vi "Demo_PlotMusic.vi"() -> ()   [LabVIEW 2021, in "RocketPlotDemo.lvlib"]
uses:
  Demo/RocketPlotDemo.lvlib
  TypeDefs/plot load data V2.ctl
  TypeDefs/plot properties V2.ctl
  TypeDefs/plot attributes V2.ctl
  TypeDefs/Plot scale axis properties.ctl
  TypeDefs/Plot general properties.ctl
  Classes/RocketPlotHandle/SubVIs/Init Options.ctl
  TypeDefs/TimeZone.ctl
  <vilib>/sound2/lvsound2.llb/Sampling Mode.ctl
  Classes/RocketPlotPanel/RocketPlotPanel.lvclass/RocketPlotPanel.ctl
  Classes/BjusticePlotHandle/BjusticePlotHandle.lvclass/BjusticePlotHandle.ctl
  4dfea61d-788a-4186-b191-4cde70d6fed2.vi
  966c8643-725a-46bd-9dd0-b91467cf4ddd.vi
  eb0507fd-03f2-4275-8513-22fa9a77d05c.vi
  2cc444ce-eb93-4e53-95b9-bbf802b1ec09.vi
  0323ff41-b8ad-4ed8-8c31-07cadd3001fa.vi
  44d01159-0067-4c41-b020-b8d23d8c44ab.vi
  286f873d-ace6-4cc1-b7d0-d8c3bbebe2d8.vi
  d8c1f50c-a031-4c7b-bbc9-5a9a3e4568ff.vi
  d49b8d8d-7917-4e09-824a-362aaf82a6cf.vi
  35cc1419-e3af-44ec-a6f0-6af3754db062.vi
  Classes/RocketPlotPanel/Read RocketPlotHandle.vi
  Classes/BjusticePlotHandle/Read sub names.vi
  Classes/BjusticePlotHandle/Read time to plot.vi
  <userlib>/bjustice/Ring Buffer for Time Series Data Strict Accessor/Unix time epoch/Unix_Epoch_in_Labview.vi
  0323ff41-b8ad-4ed8-8c31-07cadd3001fa.vi/4c2a6c61-f100-483c-8a49-51e57025a24c.vi
  0323ff41-b8ad-4ed8-8c31-07cadd3001fa.vi/e57bc314-87c7-4952-9bc8-929005dac297.vi
  44d01159-0067-4c41-b020-b8d23d8c44ab.vi/4c2a6c61-f100-483c-8a49-51e57025a24c.vi
  44d01159-0067-4c41-b020-b8d23d8c44ab.vi/e57bc314-87c7-4952-9bc8-929005dac297.vi
  <userlib>/bjustice/Ring Buffer for Time Series Data/API Poly.vi
  <userlib>/bjustice/Ring Buffer for Time Series Data/API/Write Array.vi
  d8c1f50c-a031-4c7b-bbc9-5a9a3e4568ff.vi/f2df9050-0eef-46c6-aff6-3ce3a8893ea5.vi
  35cc1419-e3af-44ec-a6f0-6af3754db062.vi/f2df9050-0eef-46c6-aff6-3ce3a8893ea5.vi
  <userlib>/bjustice/Ring Buffer for Time Series Data/SubVIs/Split Values Array.vi
  <userlib>/bjustice/Ring Buffer for Time Series Data/SubVIs/Replace Values Array Multiple Timestamps.vi
  d8c1f50c-a031-4c7b-bbc9-5a9a3e4568ff.vi/f2df9050-0eef-46c6-aff6-3ce3a8893ea5.vi/63c583a5-c20f-4aba-9c90-661423dee4c4.vi
  d8c1f50c-a031-4c7b-bbc9-5a9a3e4568ff.vi/f2df9050-0eef-46c6-aff6-3ce3a8893ea5.vi/52385341-3d9c-45d2-aff5-e082a4793eb1.vi
  d8c1f50c-a031-4c7b-bbc9-5a9a3e4568ff.vi/f2df9050-0eef-46c6-aff6-3ce3a8893ea5.vi/37f29efa-f142-46b1-a185-f0098a95fbb6.vi
  d8c1f50c-a031-4c7b-bbc9-5a9a3e4568ff.vi/f2df9050-0eef-46c6-aff6-3ce3a8893ea5.vi/84b3d231-9afe-4b6e-afae-e0be43a31e4e.vi
  d8c1f50c-a031-4c7b-bbc9-5a9a3e4568ff.vi/f2df9050-0eef-46c6-aff6-3ce3a8893ea5.vi/c726271c-fc36-4bb7-8553-8945ec40c1cd.vi
  d8c1f50c-a031-4c7b-bbc9-5a9a3e4568ff.vi/f2df9050-0eef-46c6-aff6-3ce3a8893ea5.vi/a7b1d944-dc88-46f5-9d3e-305d46bbe1f6.vi
  d8c1f50c-a031-4c7b-bbc9-5a9a3e4568ff.vi/f2df9050-0eef-46c6-aff6-3ce3a8893ea5.vi/8abc4a6e-a1d2-4e85-879b-517e0ab55733.vi
  d8c1f50c-a031-4c7b-bbc9-5a9a3e4568ff.vi/f2df9050-0eef-46c6-aff6-3ce3a8893ea5.vi/bd347357-b475-4a03-9ac5-3b85ef11aecc.vi
  d8c1f50c-a031-4c7b-bbc9-5a9a3e4568ff.vi/f2df9050-0eef-46c6-aff6-3ce3a8893ea5.vi/391b36e9-a702-45e4-9499-3914f8833a58.vi
  d8c1f50c-a031-4c7b-bbc9-5a9a3e4568ff.vi/f2df9050-0eef-46c6-aff6-3ce3a8893ea5.vi/44155b33-c915-49ce-9e44-a66693aa70dd.vi
  d8c1f50c-a031-4c7b-bbc9-5a9a3e4568ff.vi/f2df9050-0eef-46c6-aff6-3ce3a8893ea5.vi/36977d53-dbe0-4dbc-b2ac-3dea4345b868.vi
  35cc1419-e3af-44ec-a6f0-6af3754db062.vi/f2df9050-0eef-46c6-aff6-3ce3a8893ea5.vi/63c583a5-c20f-4aba-9c90-661423dee4c4.vi
  35cc1419-e3af-44ec-a6f0-6af3754db062.vi/f2df9050-0eef-46c6-aff6-3ce3a8893ea5.vi/52385341-3d9c-45d2-aff5-e082a4793eb1.vi
  35cc1419-e3af-44ec-a6f0-6af3754db062.vi/f2df9050-0eef-46c6-aff6-3ce3a8893ea5.vi/37f29efa-f142-46b1-a185-f0098a95fbb6.vi
  35cc1419-e3af-44ec-a6f0-6af3754db062.vi/f2df9050-0eef-46c6-aff6-3ce3a8893ea5.vi/84b3d231-9afe-4b6e-afae-e0be43a31e4e.vi
  35cc1419-e3af-44ec-a6f0-6af3754db062.vi/f2df9050-0eef-46c6-aff6-3ce3a8893ea5.vi/c726271c-fc36-4bb7-8553-8945ec40c1cd.vi
  35cc1419-e3af-44ec-a6f0-6af3754db062.vi/f2df9050-0eef-46c6-aff6-3ce3a8893ea5.vi/a7b1d944-dc88-46f5-9d3e-305d46bbe1f6.vi
  35cc1419-e3af-44ec-a6f0-6af3754db062.vi/f2df9050-0eef-46c6-aff6-3ce3a8893ea5.vi/8abc4a6e-a1d2-4e85-879b-517e0ab55733.vi
  35cc1419-e3af-44ec-a6f0-6af3754db062.vi/f2df9050-0eef-46c6-aff6-3ce3a8893ea5.vi/bd347357-b475-4a03-9ac5-3b85ef11aecc.vi
  35cc1419-e3af-44ec-a6f0-6af3754db062.vi/f2df9050-0eef-46c6-aff6-3ce3a8893ea5.vi/391b36e9-a702-45e4-9499-3914f8833a58.vi
  35cc1419-e3af-44ec-a6f0-6af3754db062.vi/f2df9050-0eef-46c6-aff6-3ce3a8893ea5.vi/44155b33-c915-49ce-9e44-a66693aa70dd.vi
  35cc1419-e3af-44ec-a6f0-6af3754db062.vi/f2df9050-0eef-46c6-aff6-3ce3a8893ea5.vi/36977d53-dbe0-4dbc-b2ac-3dea4345b868.vi
  <userlib>/bjustice/Ring Buffer for Time Series Data/SubVIs/Enforce array size multiple timestamps.vi
  Classes/BjusticePlotHandle/BjusticePlotHandle.lvclass
  C:/Users/bjustice/Documents/GitHub/BluePlot/Source/Classes/RocketPlotHandle/RocketPlotHandle.lvclass
  Classes/RocketPlotPanel/RocketPlotPanel.lvclass
  C:/Program Files/National Instruments/LabVIEW 2021/vi.lib/IlluminatedG/IG OOPanel/OOPanel/Panel/Panel.lvclass
  <vilib>/sound2/lvsound2.llb/Sound File Info (path).vi
  <vilib>/sound2/lvsound2.llb/Sound File Read Open.vi
  <vilib>/sound2/lvsound2.llb/Sound Output Set Volume (Single).vi
  Classes/RocketPlotHandle/Load PlotConfig.vi
  Classes/RocketPlotHandle/Get PlotConfig.vi
  <vilib>/sound2/lvsound2.llb/Sound File Read (DBL).vi
  <vilib>/Utility/error.llb/Error Cluster From Error Code.vi
  <vilib>/sound2/lvsound2.llb/Sound Output Write (DBL).vi
  Classes/RocketPlotHandle/RocketPlotHandle.lvclass
  RocketPlot.lvlib
  <userlib>/bjustice/Ring Buffer for Time Series Data Strict Accessor/Ring Buffer Strict Accessor.lvlib
  <vilib>/IlluminatedG/IG OOPanel/OOPanel/Manager/Manager.lvclass
  C:/Users/bjustice/Documents/GitHub/BluePlot/Source/Classes/BjusticePlotHandle/BjusticePlotHandle.lvclass
panel:
  in  "volume":dbl=100.0
  out "total number of samples/ch":u32
  out "Current Iteration":i32
  out "Current Data":waveform(dbl)[](graph)
  in  "load config":bool
  in  "get config":bool
  out "time to plot":dbl
  out "Subscribed names":i32(listbox)
  in  "Plot config":T1={"plots"=[], "X-axis"={"Name Label.Text"="", "Style"=0, "Tick Colors:Minor Tick Color"=0, "Tick Colors:Tick Color"=0, "Marker Colors:Text Color"=0, "Grid Colors:Major Color"=0, "Grid Colors:Minor Color"=0, "Mapping Mode"=0, "Flipped"=FALSE, "Name Label.Visible"=FALSE, "Name Label.Text Colors:Text Color"=0, "Scale Fit"=0, "Range:Maximum"=0.0, "Range:Minimum"=0.0, "Offset and Multiplier:Multiplier"=0.0, "Offset and Multiplier:Offset"=0.0, "Name Label.Font:Size"=0, "Marker.Font:Size"=0, "Uniform Marker Spacing?"=TRUE, "Format String"=""}, "Y-axes"=[], "General"={"Title"="", "Time to Plot"=1800.0, "Title.Visible"=FALSE, "Sidebar.Visible"=FALSE, "Plot Area:Colors:BG Color"=0, "X Scale.Plot Name"="", "X Scale.Use Plot Name"=FALSE}} {"General"."Time to Plot" format="%<%M:%S>t"}
  # "Documentation and user guide:"
  # "https://github.com/justiceb/BluePlot/blob/main/README.md"
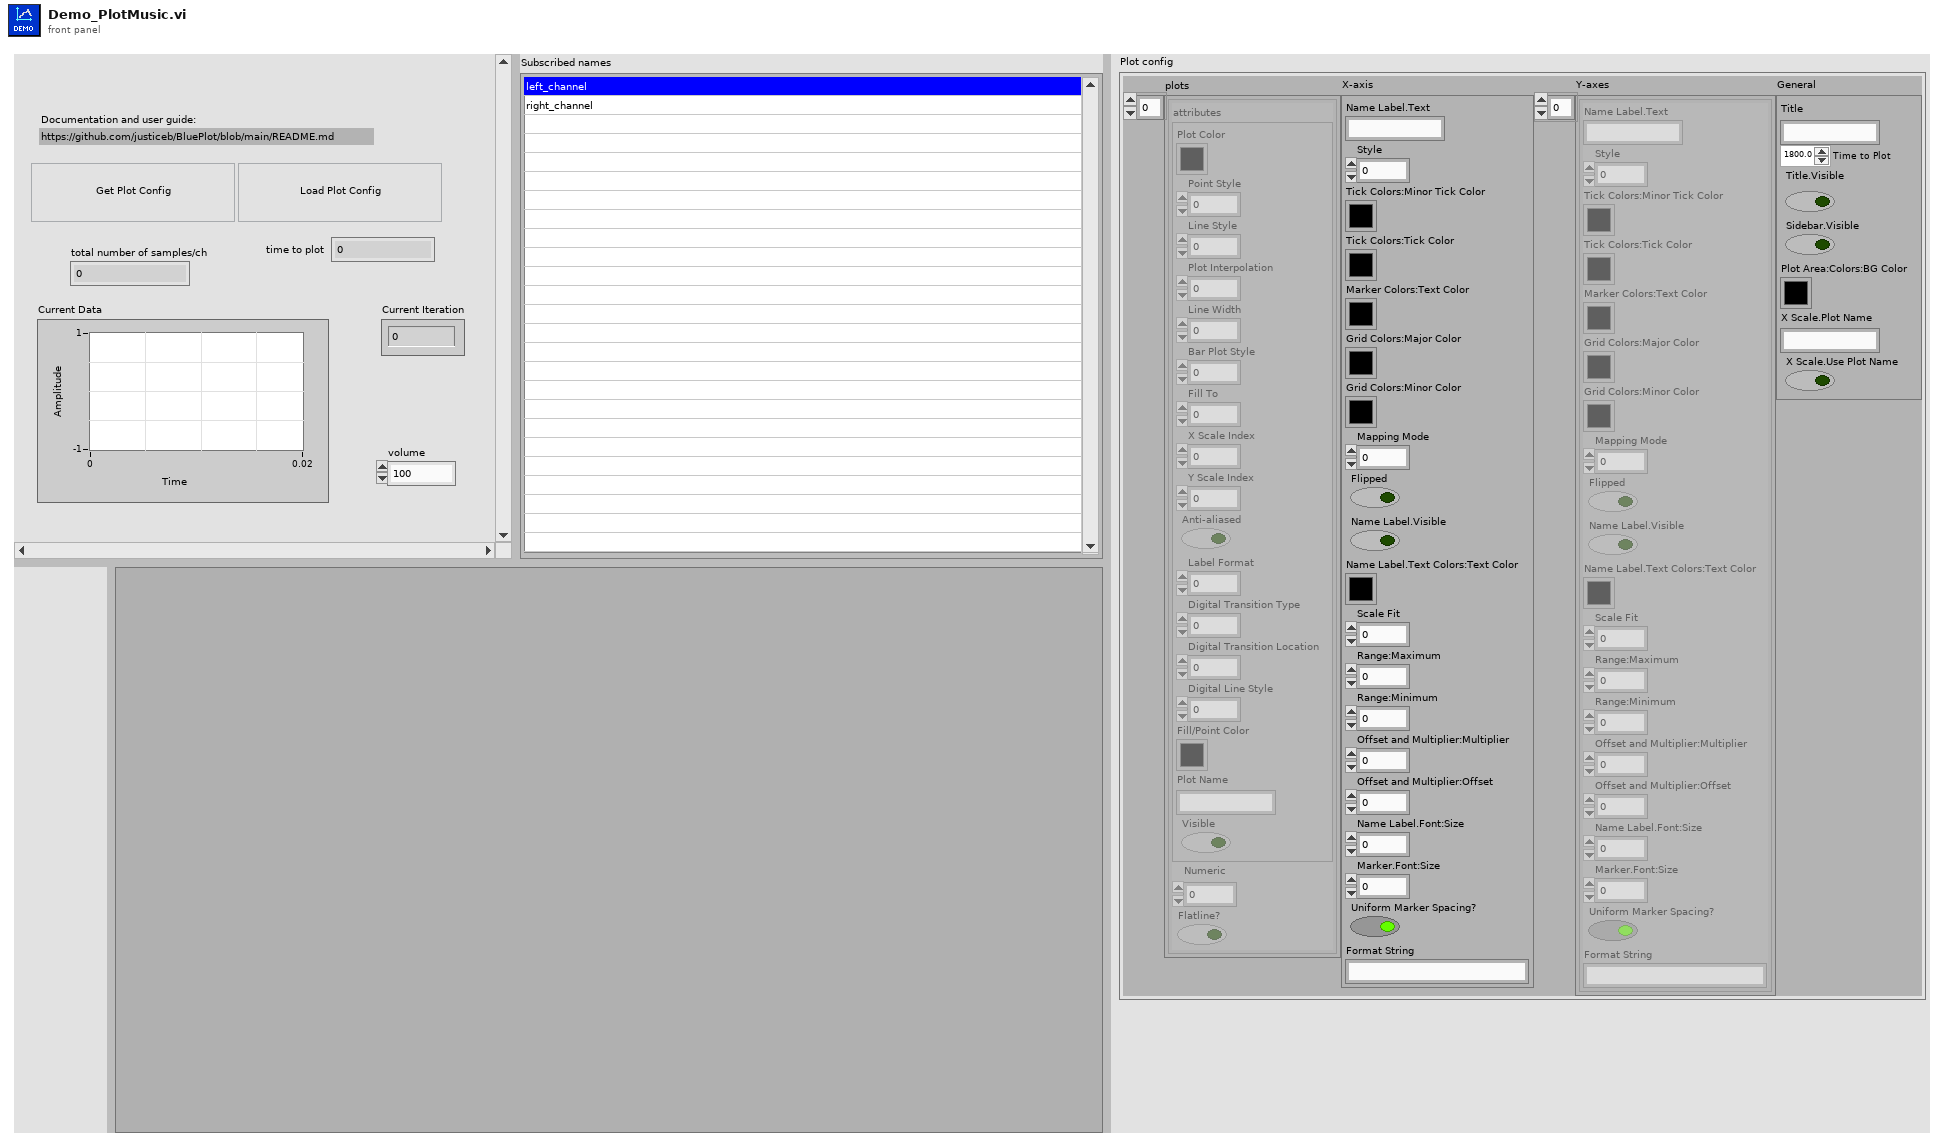
[diagram p1: front panel]
types:
  T1 = typedef "RocketPlot.lvlib/plot load data V2.ctl" = cluster{"plots":T2[], "X-axis":T4, "Y-axes":T4[], "General":T5}
  T2 = typedef "RocketPlot.lvlib/plot properties V2.ctl" = cluster{"attributes":T3, "Numeric":dbl, "Flatline?":bool}
  T3 = typedef "RocketPlot.lvlib/plot attributes V2.ctl" = cluster{"Plot Color":u32, "Point Style":u8, "Line Style":u8, "Plot Interpolation":u8, "Line Width":u8, "Bar Plot Style":u8, "Fill To":i16, "X Scale Index":u32, "Y Scale Index":u32, "Anti-aliased":bool, "Label Format":u8, "Digital Transition Type":u8, "Digital Transition Location":u8, "Digital Line Style":u8, "Fill/Point Color":u32, "Plot Name":string, "Visible":bool}
  T4 = typedef "RocketPlot.lvlib/Plot scale axis properties.ctl" = cluster{"Name Label.Text":string, "Style":u8, "Tick Colors:Minor Tick Color":u32, "Tick Colors:Tick Color":u32, "Marker Colors:Text Color":u32, "Grid Colors:Major Color":u32, "Grid Colors:Minor Color":u32, "Mapping Mode":u8, "Flipped":bool, "Name Label.Visible":bool, "Name Label.Text Colors:Text Color":u32, "Scale Fit":u8, "Range:Maximum":dbl, "Range:Minimum":dbl, "Offset and Multiplier:Multiplier":dbl, "Offset and Multiplier:Offset":dbl, "Name Label.Font:Size":u32, "Marker.Font:Size":u32, "Uniform Marker Spacing?":bool, "Format String":string}
  T5 = typedef "RocketPlot.lvlib/Plot general properties.ctl" = cluster{"Title":string, "Time to Plot":dbl, "Title.Visible":bool, "Sidebar.Visible":bool, "Plot Area:Colors:BG Color":u32, "X Scale.Plot Name":string, "X Scale.Use Plot Name":bool}
  T6 = typedef "Sampling Mode.ctl" = i32
  T7 = typedef "RocketPlotHandle.lvclass/Init Options.ctl" = cluster{"UI visible?":bool, "Update rate (ms)":u32, "Sidebar.Visible":bool, "time to plot (init)":dbl, "time to plot (max)":dbl, "config file start path":path, "Title.Visible":bool, "Title":string, "TimeZone":T8}
  T8 = typedef "RocketPlot.lvlib/TimeZone.ctl" = enum16{"UTC", "Local"}
  T9 = typedef "Sound Data Format.ctl" = cluster{"sample rate (S/s)":dbl, "number of channels":i32, "bits per sample":i32}
  T10 = typedef "Ring Buffer Strict Accessor.lvlib/RingBufferHandle.ctl" = cluster{"Ring buffer DVR":refnum<data-value>, "Data Type":T11, "Size(s)":i32[], "Endianess":T12, "Buffer Size (#timestamps) [init]":i32}
  T11 = typedef "Ring Buffer Strict Accessor.lvlib/DataType.ctl" = enum16{"uint8", "uint16", "uint32", "uint64", "int8", "int16", "int32", "int64", "float", "double", "extended"}
  T12 = typedef "Ring Buffer Strict Accessor.lvlib/Endianess.ctl" = enum16{"big-endian", "little-endian"}
  T13 = typedef "Sound File Refnum.ctl" = refnum<file>
  T14 = typedef "Sound Output Task ID.ctl" = u32
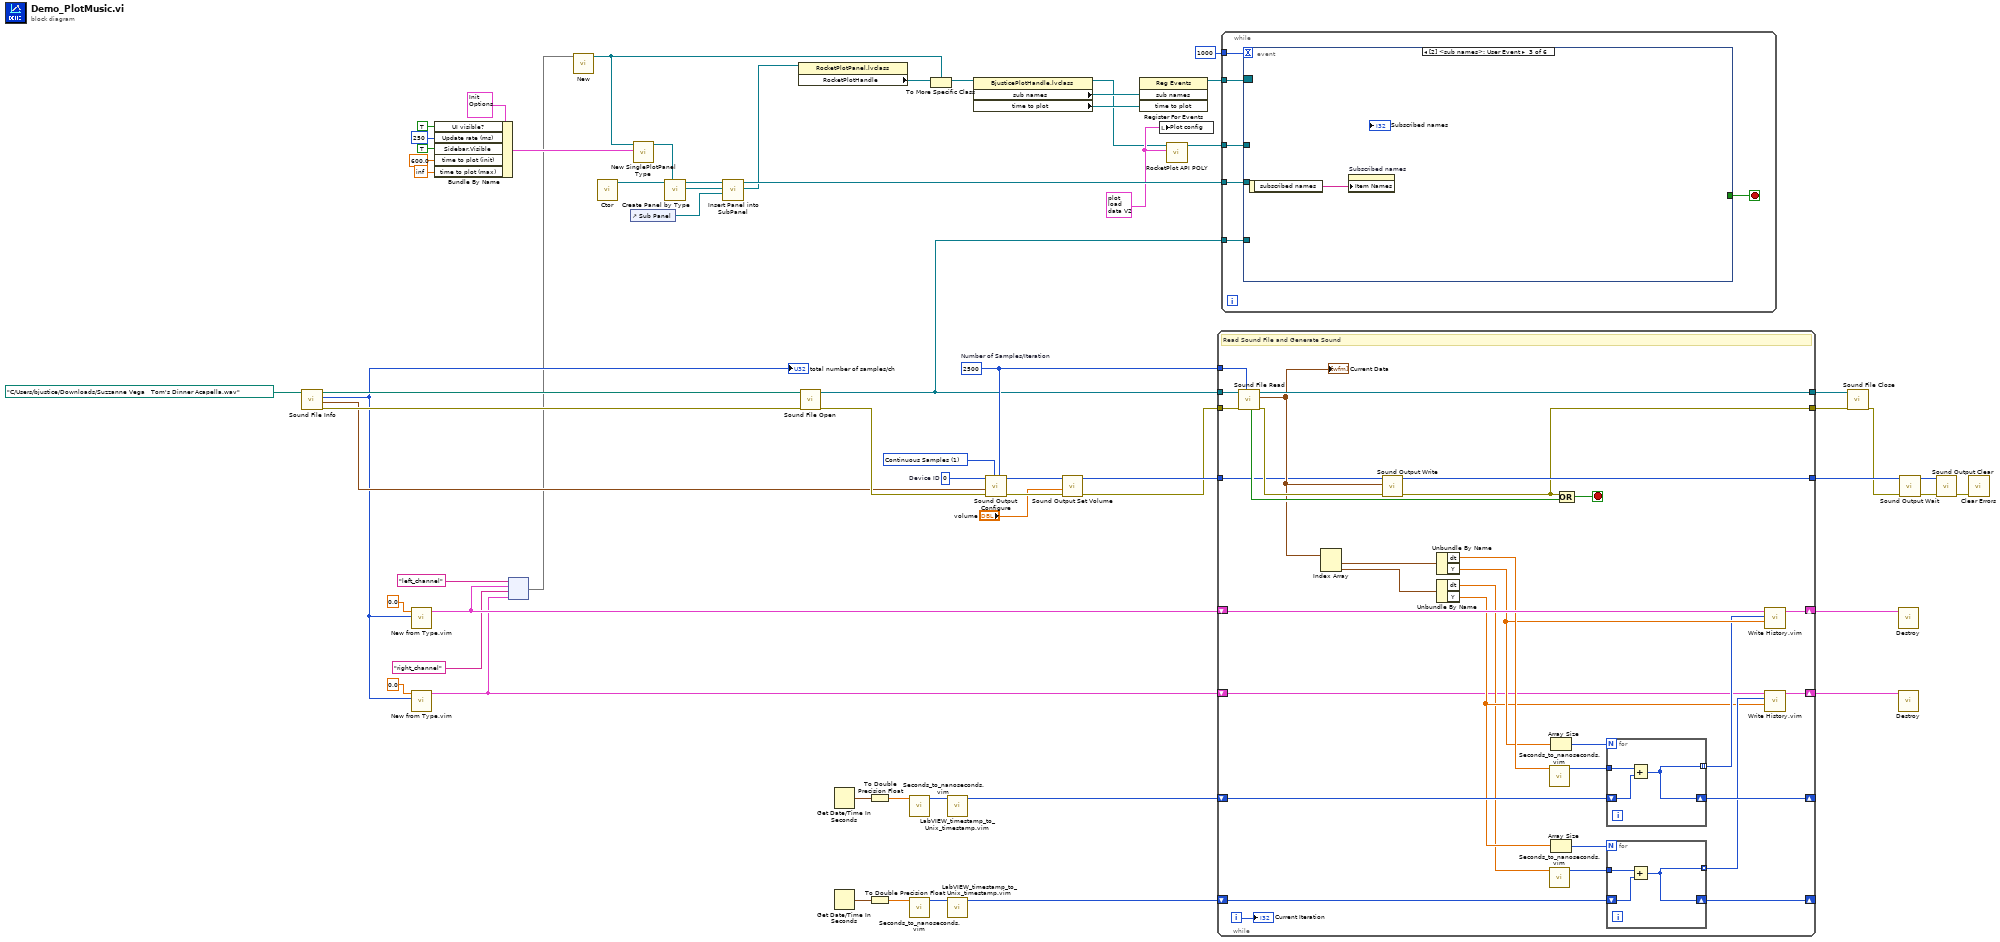
[diagram p0: block diagram]
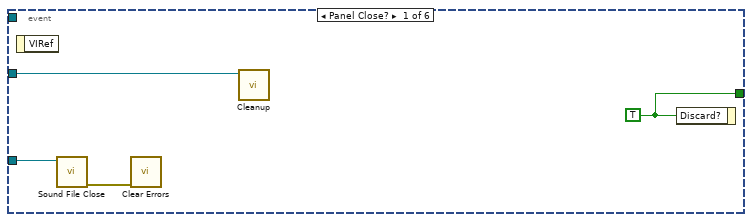
[diagram p2: hidden frame]
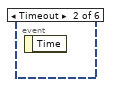
[diagram p3: hidden frame]
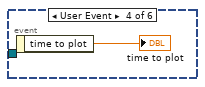
[diagram p4: hidden frame]
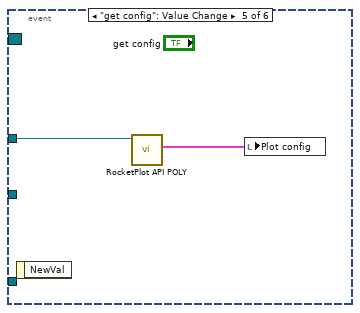
[diagram p5: hidden frame]
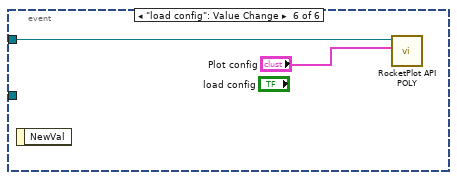
[diagram p6: hidden frame]
diagram:
  w23 = u32 0  # Device ID
  w22 = T6 1 items=["Finite Samples", "Continuous Samples"] ("sample mode")
  w24 = T1 {"plots"=[{"attributes"={"Plot Color"=16711680, "Point Style"=0, "Line Style"=0, "Plot Interpolation"=2, "Line Width"=0, "Bar Plot Style"=0, "Fill To"=-1, "X Scale Index"=0, "Y Scale Index"=0, "Anti-aliased"=FALSE, "Label Format"=3, "Digital Transition Type"=0, "Digital Transition Location"=2, "Digital Line Style"=1, "Fill/Point Color"=16711680, "Plot Name"="left_channel", "Visible"=TRUE}, "Numeric"=0.0, "Flatline?"=FALSE}, {"attributes"={"Plot Color"=4387583, "Point Style"=0, "Line Style"=0, "Plot Interpolation"=2, "Line Width"=0, "Bar Plot Style"=0, "Fill To"=-1, "X Scale Index"=0, "Y Scale Index"=1, "Anti-aliased"=FALSE, "Label Format"=3, "Digital Transition Type"=0, "Digital Transition Location"=2, "Digital Line Style"=1, "Fill/Point Color"=4387583, "Plot Name"="right_channel", "Visible"=TRUE}, "Numeric"=0.0, "Flatline?"=FALSE}, {"attributes"={"Plot Color"=16722671, "Point Style"=0, "Line Style"=0, "Plot Interpolation"=2, "Line Width"=5, "Bar Plot Style"=0, "Fill To"=-1, "X Scale Index"=0, "Y Scale Index"=0, "Anti-aliased"=FALSE, "Label Format"=3, "Digital Transition Type"=0, "Digital Transition Location"=2, "Digital Line Style"=1, "Fill/Point Color"=16722671, "Plot Name"="", "Visible"=TRUE}, "Numeric"=0.0, "Flatline?"=FALSE}], "X-axis"={"Name Label.Text"="Time (s)", "Style"=0, "Tick Colors:Minor Tick Color"=16777216, "Tick Colors:Tick Color"=3684408, "Marker Colors:Text Color"=16448250, "Grid Colors:Major Color"=3684408, "Grid Colors:Minor Color"=16777216, "Mapping Mode"=0, "Flipped"=FALSE, "Name Label.Visible"=TRUE, "Name Label.Text Colors:Text Color"=16448250, "Scale Fit"=2, "Range:Maximum"=3867076442.0, "Range:Minimum"=3867076433.0, "Offset and Multiplier:Multiplier"=1.0, "Offset and Multiplier:Offset"=0.0, "Name Label.Font:Size"=15, "Marker.Font:Size"=15, "Uniform Marker Spacing?"=TRUE, "Format String"="%<%H:%M:%S>T"}, "Y-axes"=[{"Name Label.Text"="Left Axis", "Style"=0, "Tick Colors:Minor Tick Color"=16777216, "Tick Colors:Tick Color"=3684408, "Marker Colors:Text Color"=16448250, "Grid Colors:Major Color"=3684408, "Grid Colors:Minor Color"=16777216, "Mapping Mode"=0, "Flipped"=FALSE, "Name Label.Visible"=FALSE, "Name Label.Text Colors:Text Color"=16448250, "Scale Fit"=2, "Range:Maximum"=0.5, "Range:Minimum"=-0.5, "Offset and Multiplier:Multiplier"=1.0, "Offset and Multiplier:Offset"=0.0, "Name Label.Font:Size"=15, "Marker.Font:Size"=15, "Uniform Marker Spacing?"=TRUE, "Format String"="%#_g"}, {"Name Label.Text"="Right Axis", "Style"=0, "Tick Colors:Minor Tick Color"=16777216, "Tick Colors:Tick Color"=3684408, "Marker Colors:Text Color"=16448250, "Grid Colors:Major Color"=3684408, "Grid Colors:Minor Color"=16777216, "Mapping Mode"=0, "Flipped"=FALSE, "Name Label.Visible"=FALSE, "Name Label.Text Colors:Text Color"=16448250, "Scale Fit"=2, "Range:Maximum"=0.5, "Range:Minimum"=-0.6000000000000001, "Offset and Multiplier:Multiplier"=1.0, "Offset and Multiplier:Offset"=0.0, "Name Label.Font:Size"=15, "Marker.Font:Size"=15, "Uniform Marker Spacing?"=TRUE, "Format String"="%#_g"}], "General"={"Title"="Title", "Time to Plot"=600.0, "Title.Visible"=TRUE, "Sidebar.Visible"=TRUE, "Plot Area:Colors:BG Color"=0, "X Scale.Plot Name"="", "X Scale.Use Plot Name"=FALSE}} ("Plot config 2")
  w56 = 2500  # Number of Samples/Iteration
  n1 = call-poly <vilib>:"Sound File Info.vi"("path"=path "C:/Users/bjustice/Downloads/Suzzanne Vega   Tom's Dinner Acapella.wav") -> ("error out"=w61:errorcluster, "sound format"=w35:T9, "total number of samples/ch"=w25:u32, "path out"=w57:path)  [unwired: 7 in]
  "total number of samples/ch" <- w25
  n2 = call "New from Type.vim"("Buffer Size (#timestamps)"=w25, "LV type (array size cannot be empty)"=0.0 ("value")) -> ("Ring Buffer"=w12:T10)  [unwired: 8 in, 1 out]
  n3 = call "New from Type.vim"("Buffer Size (#timestamps)"=w25, "LV type (array size cannot be empty)"=0.0 ("value")) -> ("Ring Buffer"=w10:T10)  [unwired: 8 in, 1 out]
  n4 = Bundle By Name(cluster=T7 {"UI visible?"=TRUE, "Update rate (ms)"=250, "Sidebar.Visible"=TRUE, "time to plot (init)"=600.0, "time to plot (max)"=inf, "config file start path"=path "", "Title.Visible"=TRUE, "Title"="Title", "TimeZone"=enum."Local"} ("Init options"), "UI visible?"=TRUE, "Update rate (ms)"=u32 250, "Sidebar.Visible"=TRUE ("visible sidebar?"), "time to plot (init)"=600.0, "time to plot (max)"=inf) -> (w45:T7)
  n5 = node("left_channel" ("Name (Read/Add)"), w12, "right_channel" ("Name (Read/Add)"), w10) -> (w9:map{string, T10})
  n6 = call <userlib>:"New.vi"("ChannelMap"=w9) -> ("StokePlotHandle out"=w5:refnum<class "BjusticePlotHandle.lvclass">)  [unwired: 9 in, 1 out]
  n7 = call <vilib>:"Ctor.vi"() -> ("Manager out"=w46:refnum<class "Manager.lvclass">)  [unwired: 10 in, 1 out]
  n8 = control-ref of="Sub Panel"() -> (w42:refnum<vi>)
  n9 = call "New SinglePlotPanel Type.vi"("Init options"=w45, "BluePlotHandle"=w5) -> ("SinglePlotPanel out"=w44:refnum<class "RocketPlotPanel.lvclass">)  [unwired: 8 in, 1 out]
  n10 = call <vilib>:"Create Panel by Type.vi"("Panel Type"=w44, "Manager in"=w46) -> ("Panel"=w41:refnum<class "RocketPlotPanel.lvclass">, "Manager out"=w43:refnum<class "Manager.lvclass">)  [unwired: 7 in, 1 out]
  n11 = call <vilib>:"Insert Panel into SubPanel.vi"("SubPanel"=w42, "Panel In"=w41, "Manager in"=w43) -> ("Panel"=w6:refnum<class "RocketPlotPanel.lvclass">, "Manager out"=w40:refnum<class "Manager.lvclass">)  [unwired: 6 in, 1 out]
  n12 = property class="RocketPlotPanel.lvclass"(reference=w6) -> ("RocketPlotHandle"=w8:refnum<class "RocketPlotHandle.lvclass">)  [unwired: 1 in, 2 out]
  n13 = call-poly <vilib>:"Sound File Open.vi"("error in (no error)"=w61, "path"=w57) -> ("error out"=w60:errorcluster, "sound file refnum"=w26:T13)  [unwired: 8 in]
  n14 = Get Date/Time In Seconds() -> (seconds since 1Jan1904=w37:timestamp)
  n15 = Get Date/Time In Seconds() -> (seconds since 1Jan1904=w30:timestamp)
  n16 = To Double Precision Float(number=w37) -> (double precision float=w36:dbl)
  n17 = To Double Precision Float(number=w30) -> (double precision float=w31:dbl)
  n18 = call "Seconds_to_nanoseconds.vim"("timestamp (seconds)"=w36) -> ("timestamp (nanoseconds)"=w39:u64)  [unwired: 10 in]
  n19 = call "Seconds_to_nanoseconds.vim"("timestamp (seconds)"=w31) -> ("timestamp (nanoseconds)"=w29:u64)  [unwired: 10 in]
  n20 = To More Specific Class(target class=w5, reference=w8) -> (specific class reference=w7:refnum<class "BjusticePlotHandle.lvclass">)  [unwired: 1 in, 1 out]
  n21 = call "LabVIEW_timestamp_to_Unix_timestamp.vim"("LabVIEW timestamp (nanoseconds)"=w39) -> ("Unix timestamp (nanoseconds)"=w33:u64)  [unwired: 10 in]
  n22 = call "LabVIEW_timestamp_to_Unix_timestamp.vim"("LabVIEW timestamp (nanoseconds)"=w29) -> ("Unix timestamp (nanoseconds)"=w32:u64)  [unwired: 10 in]
  n23 = property class="BjusticePlotHandle.lvclass"(reference=w7) -> (reference out=w2:refnum<class "BjusticePlotHandle.lvclass">, "sub names"=w4:refnum<user-event>, "time to plot"=w3:refnum<user-event>)  [unwired: 1 in, 1 out]
  n24 = call <vilib>:"Sound Output Configure.vi"("number of samples/ch"=w56, "sample mode"=w22, "error in (no error)"=w60, "sound format"=w35, "device ID"=w23) -> ("error out"=w17:errorcluster, "task ID"=w18:T14)  [unwired: 5 in]
  n25 = call-poly <vilib>:"Sound Output Set Volume.vi"("error in (no error)"=w17, "volume"="volume", "task ID"=w18) -> ("error out"=w15:errorcluster, "task ID out"=w16:T14)  [unwired: 7 in]
  n26 = register-events(w4, w3) -> (reference out=w1:refnum<event-registration>)  [unwired: 2 in, 1 out]
  n27 = local write "Plot config"(w24) -> ()
  n28 = call-poly "RocketPlot API POLY.vi"("Plot config"=w24, "BluePlotHandle in"=w2) -> ("BluePlotHandle out"=w48:refnum<class "BjusticePlotHandle.lvclass">)  [unwired: 8 in, 1 out]
  n29 = while {
    tunnel: w56 -> [w87]
    tunnel: w26 -> [w93]
    tunnel: [w91] -> w63
    tunnel: w15 -> [w94]
    tunnel: [w86] -> w62
    tunnel: [w95] -> w59
    shift-right: [w76] -> _
    shift-left: w33 -> [w78]
    shift-right: [w75] -> _
    shift-left: w32 -> [w73]
    shift-right: [w66] -> w28
    shift-left: w12 -> [w84]
    shift-right: [w65] -> w27
    shift-left: w10 -> [w68]
    tunnel: w16 -> [w64]
    i -> [w92]
    stop <- w88 stop-if-true
    # "Read Sound File and Generate Sound"
    n30 = call-poly <vilib>:"Sound File Read.vi"("number of samples/ch (-1: all)"=w87, "error in (no error)"=w94, "sound file refnum"=w93) -> ("error out"=w90:errorcluster, "data"=w85:waveform(dbl)[], "sound file refnum out"=w91:T13, "end of file?"=w89:bool)  [unwired: 4 in, 1 out]
    "Current Data" <- w85
    n31 = Index Array(array=w85) -> (element #1=w83:waveform(dbl), element #2=w67:waveform(dbl))  [unwired: 2 in]
    n32 = call-poly <vilib>:"Sound Output Write.vi"("error in (no error)"=w90, "data"=w85, "task ID"=w64) -> ("error out"=w86:errorcluster, "task ID out"=w95:T14)  [unwired: 7 in]
    n33 = Unbundle By Name(w83) -> ("dt"=w82:dbl, "Y"=w81:dbl[])
    n34 = Unbundle By Name(w67) -> ("dt"=w69:dbl, "Y"=w70:dbl[])
    n35 = call "Seconds_to_nanoseconds.vim"("timestamp (seconds)"=w82) -> ("timestamp (nanoseconds)"=w79:u64)  [unwired: 10 in]
    n36 = call "Seconds_to_nanoseconds.vim"("timestamp (seconds)"=w69) -> ("timestamp (nanoseconds)"=w72:u64)  [unwired: 10 in]
    n37 = Array Size(array=w81) -> (size(s)=w80:i32)
    n38 = Array Size(array=w70) -> (size(s)=w71:i32)
    n39 = Compound Arithmetic op=OR(w86, w89) -> (w88:bool)
    n40 = for {
      N: w80 -> [_]
      tunnel: w79 -> [w98]
      shift-right: [w96] -> w76
      shift-left: w78 -> [w97]
      tunnel: [w96] -> w77 mode=indexing
      n41 = Add(x=w98, y=w97) -> (x+y=w96:u64)
    }
    n42 = for {
      N: w71 -> [_]
      tunnel: w72 -> [w101]
      shift-right: [w99] -> w75
      shift-left: w73 -> [w100]
      tunnel: [w99] -> w74 mode=indexing
      n43 = Add(x=w101, y=w100) -> (x+y=w99:u64)
    }
    n44 = call "Write History.vim"("LV DataType"=w81, "Timestamps"=w77, "Ring Buffer"=w84) -> ("Ring Buffer"=w66:T10)  [unwired: 7 in, 1 out]
    n45 = call "Write History.vim"("LV DataType"=w70, "Timestamps"=w74, "Ring Buffer"=w68) -> ("Ring Buffer"=w65:T10)  [unwired: 7 in, 1 out]
    "Current Iteration" <- w92
  }
  n46 = while {
    tunnel: w48 -> [w107]
    tunnel: 1000 ("period (ms)") -> [w105]
    tunnel: w40 -> [w104]
    tunnel: w26 -> [w103]
    tunnel: w1 -> [w102]
    stop <- w106 stop-if-true
    n47 = event shown="[2] <sub names>: User Event" {
      selector: w102 -> [_ _ _ _ _ _]
      dyn-events: _ -> [_ _ _ _ _ _]
      timeout: w105 -> [_ _ _ _ _ _]
      tunnel: w107 -> [_ _ _ _ w115 w117]
      tunnel: [w111 _ _ _ _ _] -> w106
      tunnel: w104 -> [w110 _ _ _ _ _]
      tunnel: w103 -> [w109 _ _ _ _ _]
      event Panel Close? {
        w111 = TRUE ("Discard?")
        n48 = event-data() -> ()  [unwired: 1 in, 1 out]
        n49 = call <vilib>:"Sound File Close.vi"("sound file refnum"=w109) -> ("error out"=w108:errorcluster)  [unwired: 10 in]
        n50 = call <vilib>:"Clear Errors.vi"("error in (no error)"=w108) -> ()  [unwired: 5 in, 2 out]
        n51 = call <vilib>:"Cleanup.vi"("Manager in"=w110) -> ()  [unwired: 8 in, 3 out]
        n52 = event-data("Discard?"=w111) -> ()  [unwired: 1 in, 1 out]
      }
      event Timeout {
        n53 = event-data() -> ()  [unwired: 1 in, 1 out]
      }
      event User Event {
        n54 = event-data() -> ("subscribed names"=w112:string[])  [unwired: 1 in]
        n55 = property on="Subscribed names" class="LstBox (strict)"("Item Names"=w112) -> ()  [unwired: 2 in, 2 out]
      }
      event User Event {
        n56 = event-data() -> ("time to plot"=→"time to plot":dbl)  [unwired: 1 in]
      }
      event "get config": Value Change {
        n57 = event-data() -> ()  [unwired: 1 in, 1 out]
        n58 = call-poly "RocketPlot API POLY.vi"("BluePlotHandle in"=w115) -> ("Plot config"=w114:T1)  [unwired: 8 in, 2 out]
        n59 = local write "Plot config"(w114) -> ()
      }
      event "load config": Value Change {
        n60 = event-data() -> ()  [unwired: 1 in, 1 out]
        n61 = call-poly "RocketPlot API POLY.vi"("Plot config"="Plot config", "BluePlotHandle in"=w117) -> ()  [unwired: 8 in, 2 out]
      }
    }
  }
  n62 = call <vilib>:"Sound File Close.vi"("error in (no error)"=w62, "sound file refnum"=w63) -> ("error out"=w58:errorcluster)  [unwired: 9 in]
  n63 = call <userlib>:"Destroy.vi"("Ring Buffer"=w28) -> ()  [unwired: 10 in, 1 out]
  n64 = call <userlib>:"Destroy.vi"("Ring Buffer"=w27) -> ()  [unwired: 10 in, 1 out]
  n65 = call <vilib>:"Sound Output Wait.vi"("error in (no error)"=w58, "task ID"=w59) -> ("error out"=w20:errorcluster, "task ID out"=w21:T14)  [unwired: 8 in]
  n66 = call <vilib>:"Sound Output Clear.vi"("error in (no error)"=w20, "task ID"=w21) -> ("error out"=w19:errorcluster)  [unwired: 9 in]
  n67 = call <vilib>:"Clear Errors.vi"("error in (no error)"=w19) -> ()  [unwired: 5 in, 2 out]
